vi "Diagnostics - Tool.vi"() -> ()   [LabVIEW 2025, in "Diagnostics Workspace Tool.lvlib"]
uses:
  Diagnostics Workspace Tool.lvlib
  Addon/Addon Shared/Types/Command.New.ctl
  NationalInstruments.VeriStand.SystemStorage
  SubModules/CAN-Streaming-Support/Source/Addon/Addon Shared/Types/Direction Filter.ctl
  SubModules/CAN-Streaming-Support/Source/Addon/Addon Shared/Types/Type Filter.ctl
  Workspace Shared/Types/Workspace.State.ctl
  Workspace Shared/Types/UI.Refs.ctl
  <vilib>/NI VeriStand/Display Template Support/DisplayTemplateSupport.llb/enum_Display Template Handler Minimal To Workspace.ctl
  Workspace Shared/Types/Workspace.SavedState.ctl
  <vilib>/NI VeriStand/Execution/Workspace/WorkspaceAPI.ctl
  <vilib>/NI VeriStand/Display Template Support/DisplayTemplateSupport.llb/enum_Display Template Handler Minimal To Widget Msg.ctl
  <vilib>/NI VeriStand/Execution/Workspace/SystemStateRegEventRef.ctl
  <vilib>/NI VeriStand/Execution/Workspace/Target State Info.ctl
  <vilib>/NI VeriStand/Execution/Workspace/Target State.ctl
  <vilib>/NI VeriStand/Execution/Workspace/SystemStateEventRef.ctl
  Addon/Addon Shared/Types/Protocol.ctl
  SubModules/CAN-Streaming-Support/Source/UIs/Workspace Shared/Types/Host Stream Queue Refs.ctl
  SubModules/CAN-Streaming-Support/Source/UIs/Workspace Shared/Types/Host Stream Queue Type.ctl
  SubModules/CAN-Streaming-Support/Source/UIs/Workspace Shared/Types/Host Stream Queue Command.ctl
  <vilib>/xnet/xnet.llb/XNET Frame CAN.ctl
  <vilib>/xnet/xnet.llb/XNET Frame Type CAN.ctl
  Addon/Addon Shared/Types/Transport.ctl
  SubModules/CAN-Streaming-Support/Source/UIs/Workspace Shared/Types/Host Stream Engine Parameters.ctl
  SubModules/CAN-Streaming-Support/Source/Addon/Addon Shared/Types/Filter Parameters.ctl
  Addon/Addon Shared/Types/Command.ReadDTC.ctl
  Addon/Addon Shared/Types/DTC.Descriptor.Override.ctl
  <vilib>/Utility/miscctls.llb/LVRowAndColumnUnsignedTypeDef.ctl
  <vilib>/Utility/error.llb/Trim Whitespace.vi
  <vilib>/dlg_ctls.llb/Space Constant.vi
  SubModules/CAN-Streaming-Support/Source/UIs/Workspace Shared/SubVIs/Create Host Stream Refs.vi
  SubModules/CAN-Streaming-Support/Source/UIs/Workspace Shared/SubVIs/Read Host Stream.vi
  SubModules/CAN-Streaming-Support/Source/UIs/Workspace Shared/SubVIs/Cleanup Host Stream.vi
  SubModules/CAN-Streaming-Support/Source/UIs/Workspace Shared/SubVIs/Create Bus Log File.vi
  SubModules/CAN-Streaming-Support/Source/UIs/Workspace Shared/SubVIs/Write to Bus Log File.vi
  SubModules/CAN-Streaming-Support/Source/UIs/Workspace Shared/SubVIs/Convert BIN to TXT File.vi
  SubModules/CAN-Streaming-Support/Source/UIs/Workspace Shared/SubVIs/Get Next Bus Engine State.vi
  SubModules/CAN-Streaming-Support/Source/UIs/Workspace Shared/SubVIs/Get Engine Trigger State.vi
  SubModules/CAN-Streaming-Support/Source/UIs/Workspace Shared/SubVIs/Get Next Log Engine State.vi
  <vilib>/Utility/error.llb/Trim Whitespace One-Sided.vi
  SubModules/CAN-Streaming-Support/Source/UIs/Workspace Shared/SubVIs/Process CAN Data.vi
  SubModules/CAN-Streaming-Support/Source/UIs/Workspace Shared/SubVIs/Process CAN State.vi
  SubModules/CAN-Streaming-Support/Source/UIs/Workspace Shared/SubVIs/Convert Frame Array to String Array.vi
  SubModules/CAN-Streaming-Support/Source/UIs/Workspace Shared/SubVIs/Convert Time to UTC String.vi
  <userlib>/_OpenG.lib/array/array.llb/Sort Array__ogtk.vi
  <userlib>/_OpenG.lib/array/array.llb/Sort 2D Array (String)__ogtk.vi
  <vilib>/Utility/libraryn.llb/Check if File or Folder Exists.vi
  <vilib>/Utility/libraryn.llb/Get File Extension.vi
  Addon/Addon Shared/SubVIs/Constants.vi
  <vilib>/NI VeriStand/Execution/Workspace/NI VeriStand - Get Multiple Channel Values.vi
  <vilib>/NI VeriStand/Execution/Workspace/NI VeriStand - Set Single Channel Value.vi
  Workspace Shared/Diagnostics Workspace Shared.lvlib
  APIs/Host Automation API/Diagnostics Host Automation API.lvlib
  Addon/Addon Shared/Diagnostics Addon Shared.lvlib
  <vilib>/NI VeriStand/Execution/Workspace/NI_VS Workspace ExecutionAPI.lvlib
  SubModules/CAN-Streaming-Support/Source/UIs/Workspace Shared/CAN Stream Support Workspace Shared.lvlib
  SubModules/CAN-Streaming-Support/Source/Addon/Addon Shared/CAN Stream Support Shared.lvlib
  NationalInstruments.VeriStand.ClientAPI
panel:
  out "Device":string
  in  "Tab Control":enum32{"Cmd", "Raw", "Read DTCs", "Bus Stream"}(tab)
  out "Time Stamp":timestamp
  out "Comm Connected?":bool
  in  "Send Cmd":bool
  out "VeriStand Error":i64 format="%.0x"
  out "Success?":bool
  in  "Cmd":T1
  in  "Clear Raw":bool
  in  "Send Raw":bool
  out "Raw VeriStand Error":errorcluster
  out "Raw Error Byte":u8 format="%.0x"
  in  "Response Required?":bool
  out "Raw Resp":u8[](array[numeric]) format="%.0x"
  in  "Raw Cmd":u8[](array[numeric]) format="%.0x"
  in  "DTC":u32
  in  "Status":u32
  in  "Failure":u32
  in  "Override Byte Lengths":bool
  in  "Extension":u32 format="%.0x"
  in  "Mask":u32 format="%.0x"
  in  "Mode":u32 format="%.0x"
  in  "Hex":bool=TRUE
  in  "DTCs":string(tree)
  in  "Read DTCs":bool
  in  "Reset Filter":bool
  in  "Host Filter":bool
  in  "Filter IDs":string caption="Filter IDs (format = x<ID>, comma separated, ID x0 = Bus Error)"
  in  "Clear History":bool
  in  "Type Filter":T2
  out "Table Control":string[][](table)
  in  "Enable Stream":bool
  in  "Pause":bool
  in  "Sort By ID":bool
  out "Stream Connected":bool
  out "Status":string
  in  "Direction Filter":T3
  in  "Log":bool
  in  "NIVS.Gateway IP Address":string
  in  "NIVS.System Definition Root":refnum<k24>
  in  "NIVS.Workspace Event":refnum<event-registration>
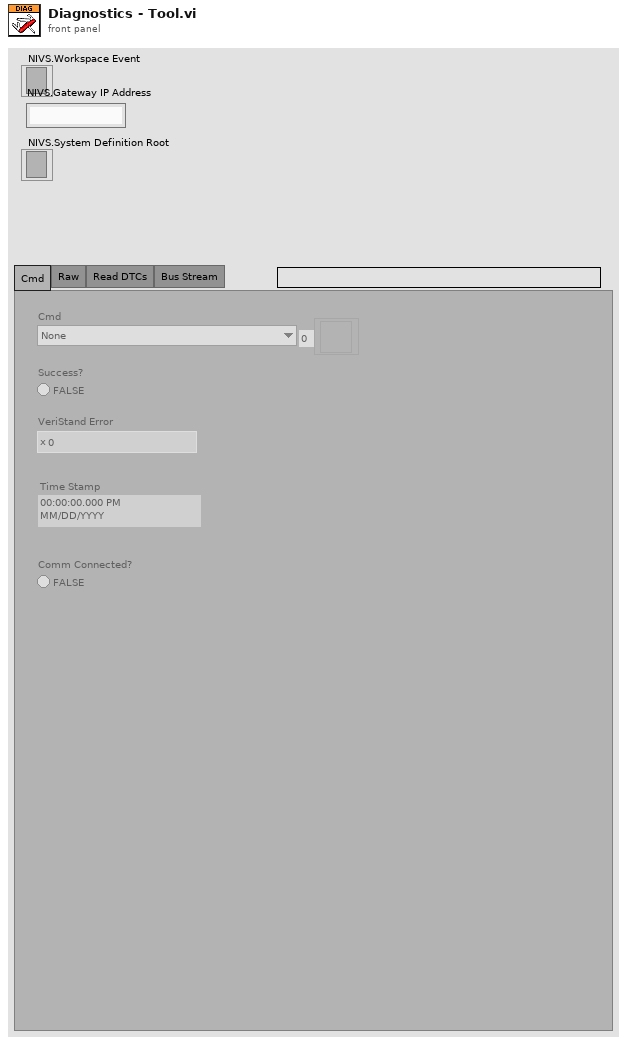
[diagram p1: front panel]
types:
  T1 = typedef "Diagnostics Addon Shared.lvlib/Command.New.ctl" = enum8{"None", "Clear Status Channels", "Read All DIDs", "Read All PIDs", "Configure and Start DPIDs", "Stop DPIDs"}
  T2 = typedef "CAN Stream Support Shared.lvlib/Type Filter.ctl" = enum16{"All", "CAN Data", "CAN Remote", "CAN Bus Error", "CAN 2.0 Data", "CAN FD Data", "CAN FD+BRS Data", "J1939 Data", "Delay", "Log Trigger", "Start Trigger"}
  T3 = typedef "CAN Stream Support Shared.lvlib/Direction Filter.ctl" = enum16{"Tx/Rx", "Rx", "Tx"}
  T4 = typedef "Diagnostics Workspace Shared.lvlib/Workspace.State.ctl" = cluster{"UI.Refs":T5, "Data.PreviousValues":dbl[], "Data.Read":string[], "CachedData.UserEvent":refnum<user-event>, "CachedData":T6, "Addon.Connected?":bool, "NIVS.SysDef":path, "NIVS.SysDefRoot":refnum<k24>, "NIVS.Workspace":T7, "NIVS.UserEventRefs":cluster{"Event Registration Refnum":refnum<event-registration>, "SystemChangeEventRef":T8, "NIVS.Workspace Event":refnum<event-registration>}, "NIVS.SystemStateRefs":T9, "NIVS.LaunchRef":refnum<user-event>, "Data.PendingChange?":bool, "Command.Channel":string, "Diagnostic Protocol":T10, "Channels.Found":bool, "Command.Connect":string, "Mode.Tool?":bool, "Stream.Qs":T11, "Transport Layer":T12}
  T5 = typedef "Diagnostics Workspace Shared.lvlib/UI.Refs.ctl" = cluster{"Cmd":refnum<vi>, "Success?":refnum<vi>, "VeriStandError":refnum<vi>, "CAN Connected?":refnum<vi>, "DTC":refnum<vi>, "Status":refnum<vi>, "Failure":refnum<vi>, "Override Byte Lengths":refnum<vi>, "Response Required?":refnum<vi>, "Send":refnum<vi>, "Clear":refnum<vi>, "Send Raw":refnum<vi>, "Read DTCs":refnum<vi>, "Raw Cmd":refnum<vi>, "Extension":refnum<vi>, "Mode":refnum<vi>, "Mask":refnum<vi>, "Hex":refnum<vi>, "Raw Resp":refnum<vi>, "Raw Error Byte":refnum<vi>, "Raw VeriStand Error":refnum<vi>, "DTCs":refnum<vi>, "Time Stamp":refnum<vi>, "Device":refnum<vi>, "Pause":refnum<vi>, "Table Control":refnum<vi>, "Sort By ID":refnum<vi>, "Streaming Connected":refnum<vi>, "Enable Stream":refnum<vi>, "CAN State":refnum<vi>, "Direction Filter":refnum<vi>, "Type Filter":refnum<vi>, "Clear History":refnum<vi>, "Filter IDs":refnum<vi>, "Filter Location":refnum<vi>, "Reset Filter":refnum<vi>, "Log":refnum<vi>}
  T6 = typedef "Diagnostics Workspace Shared.lvlib/Workspace.SavedState.ctl" = cluster{"CD Path":string, "CD IP":string}
  T7 = typedef "NI_VS Workspace ExecutionAPI.lvlib/WorkspaceAPI.ctl" = refnum<k24>
  T8 = typedef "NI_VS Workspace ExecutionAPI.lvlib/SystemStateRegEventRef.ctl" = refnum<event-registration>
  T9 = typedef "NI_VS Workspace ExecutionAPI.lvlib/SystemStateEventRef.ctl" = cluster{"CustDatRef":refnum<user-event>, "EvtRef":refnum<k27>, "Target State User Event":refnum<user-event>}
  T10 = typedef "Diagnostics Addon Shared.lvlib/Protocol.ctl" = enum16{"GMLAN", "KWP-2000", "UDS", "User-Defined"}
  T11 = typedef "CAN Stream Support Workspace Shared.lvlib/Host Stream Queue Refs.ctl" = cluster{"Cmd Q":refnum<queue>, "XNET Frames":refnum<queue>}
  T12 = typedef "Diagnostics Addon Shared.lvlib/Transport.ctl" = enum16{"ISO TP - Normal Mode", "ISO TP - Mixed Mode", "VW TP 2.0", "Diagnostics on IP", "ISO TP LIN"}
  T13 = typedef "enum_Display Template Handler Minimal To Workspace.ctl" = cluster{"Operation":enum16{"SetCustomData", "DeleteItem"}, "Data":variant}
  T14 = typedef "Diagnostics Addon Shared.lvlib/Command.ReadDTC.ctl" = cluster{"Extension":u32, "Mask":u32, "Mode/Status":u32, "Byte Lengths":T15}
  T15 = typedef "Diagnostics Addon Shared.lvlib/DTC.Descriptor.Override.ctl" = cluster{"Override":bool, "DTC":u32, "Status":u32, "Failure":u32}
  T16 = typedef "CAN Stream Support Shared.lvlib/Filter Parameters.ctl" = cluster{"ID Filters":u32[], "Direction Filter":T3, "Type Filter":T2}
  T17 = typedef "LVRowAndColumnUnsignedTypeDef.ctl" = cluster{"Row":u32, "Column":u32}
  T18 = cluster{"Event Registration Refnum":refnum<event-registration>, "SystemChangeEventRef":T8, "NIVS.Workspace Event":refnum<event-registration>}
  T19 = typedef "enum_Display Template Handler Minimal To Widget Msg.ctl" = enum16{"Stop", "LaunchConfigDialog"}
  T20 = enum8{"Enabled", "Disabled", "Disabled and Grayed Out"}
  T21 = typedef "Diagnostics Addon Shared.lvlib/HostAutomation.Ref.ctl" = cluster{"TCP Comm":T22, "DTCs":T24}
  T22 = typedef "NI STM.lvlib/TCP Connection Info.ctl" = cluster{"connection ID":refnum<k5>, "meta data":T23[]}
  T23 = typedef "NI STM.lvlib/MetaDataElement.ctl" = string
  T24 = typedef "Diagnostics Addon Shared.lvlib/DTC.Codes.ctl" = cluster{"Value.Code":dbl[], "Value.String":string[], "Value.J2012String":string[], "Status.Code":dbl[], "Status.String":string[]}
  T25 = cluster{"resp":u8[], "error code":u8, "error out":errorcluster}
  T26 = typedef "Diagnostics Addon Shared.lvlib/Command.ReadDTC.DTCs.ctl" = cluster{"Timestamp":dbl, "DTC":dbl, "J2012 String":string, "DTC String":string, "Status":dbl, "Status String":string, "Add Data":dbl}
  T27 = typedef "CAN Stream Support Workspace Shared.lvlib/Host Stream Engine Parameters.ctl" = cluster{"Host Filter":bool, "Filter Parameters":T16, "Sort By ID":bool, "Pause":bool, "Clear History":bool, "Log":bool}
  T28 = typedef "CAN Stream Support Workspace Shared.lvlib/Host Stream Data.ctl" = cluster{"Connected":bool, "Bus Data Update":bool, "Bus Data":string[][], "Bus Status":string, "Bus Warning":bool, "Log Status":string}
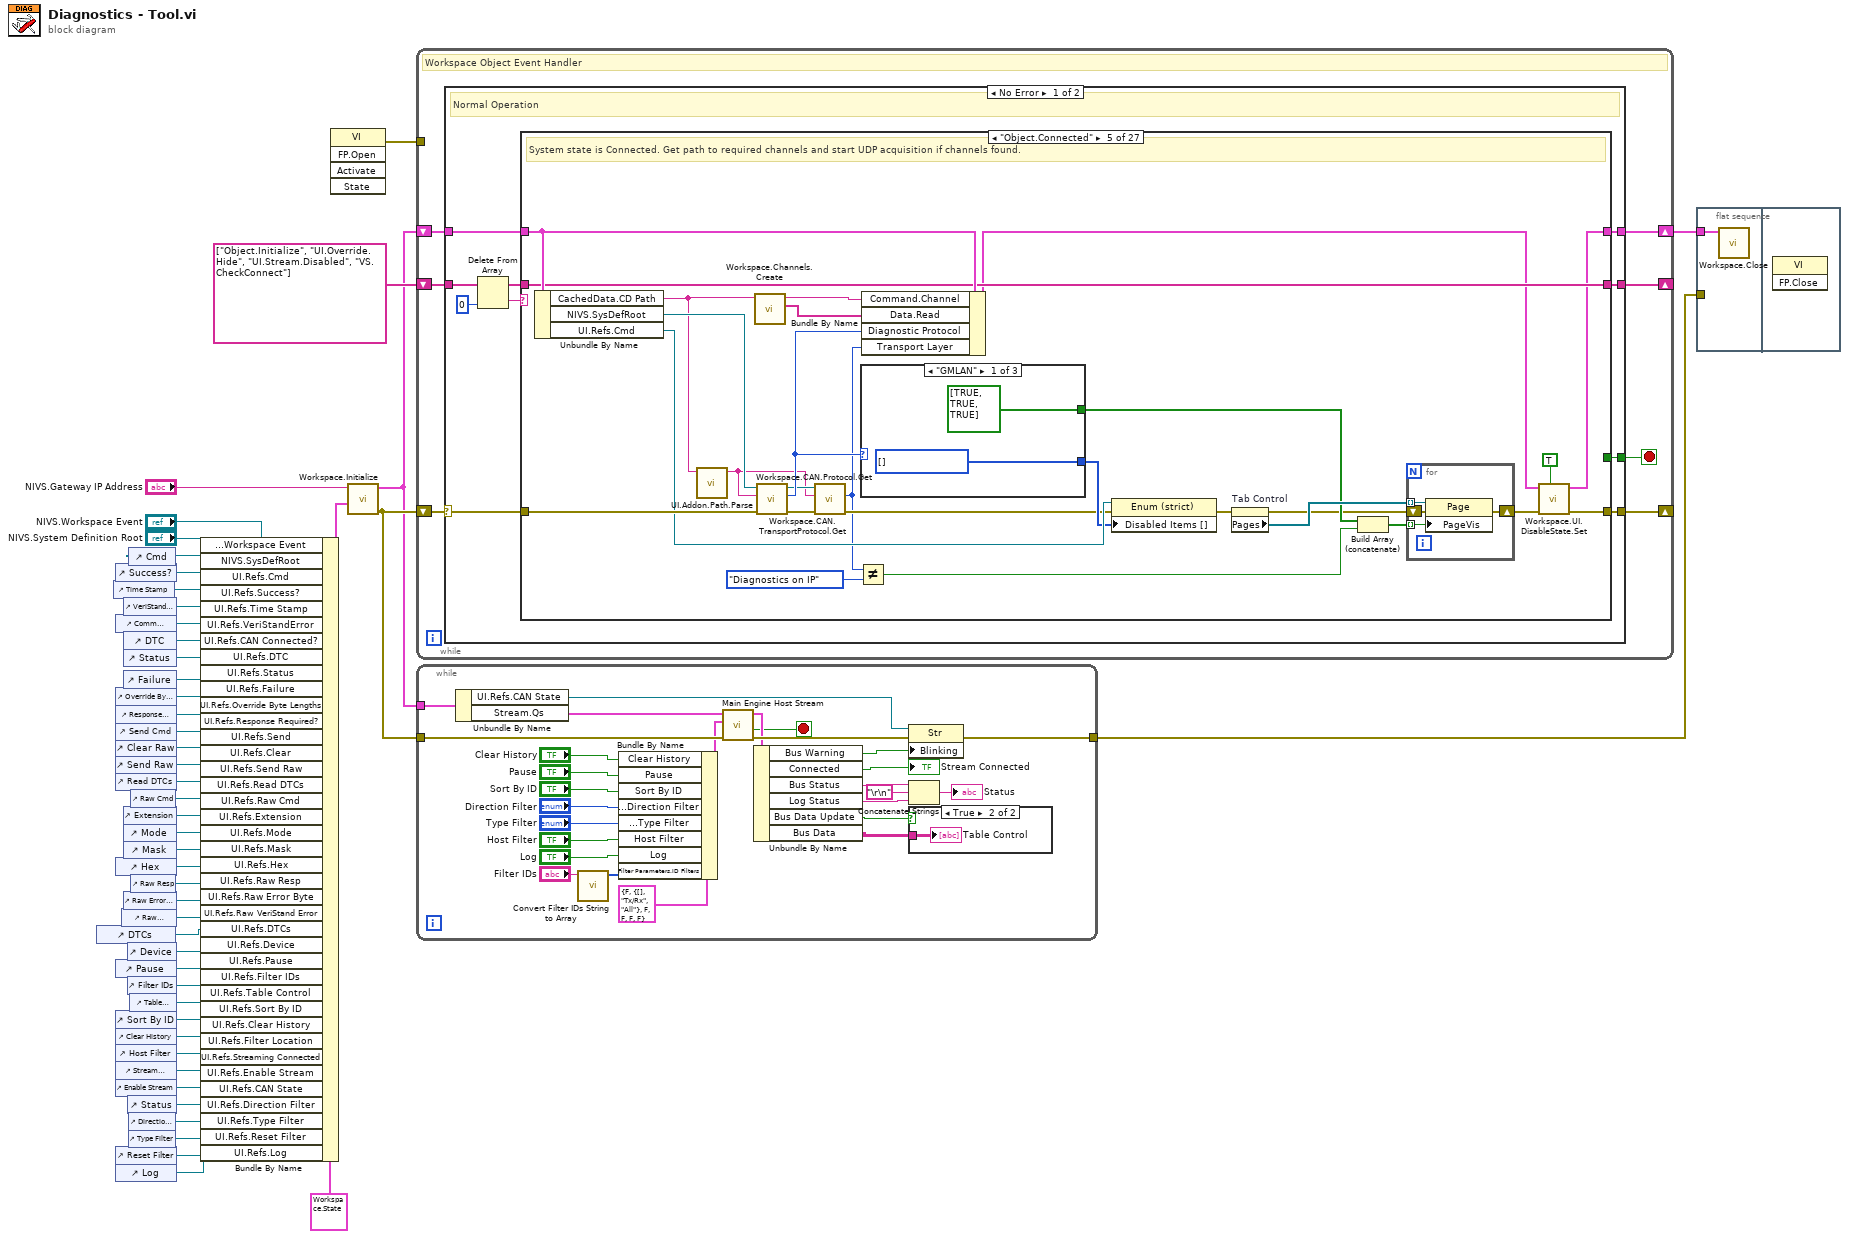
[diagram p0: block diagram]
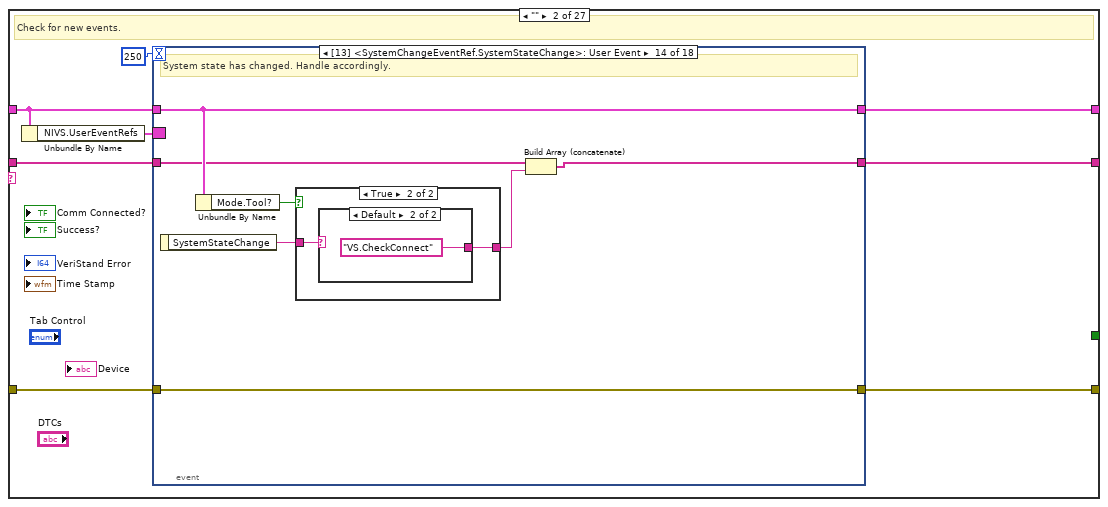
[diagram p4: hidden frame]
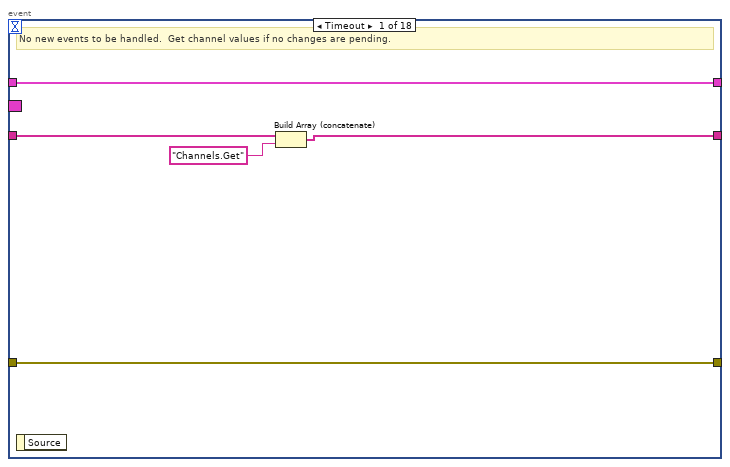
[diagram p5: hidden frame]
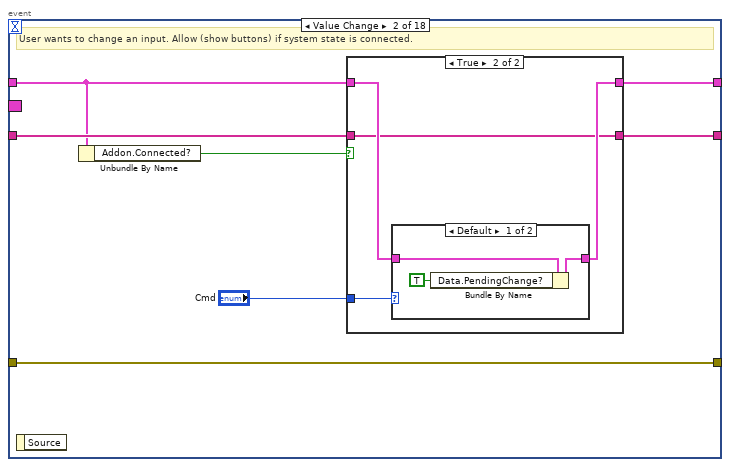
[diagram p6: hidden frame]
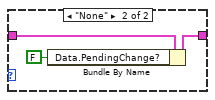
[diagram p8: hidden frame]
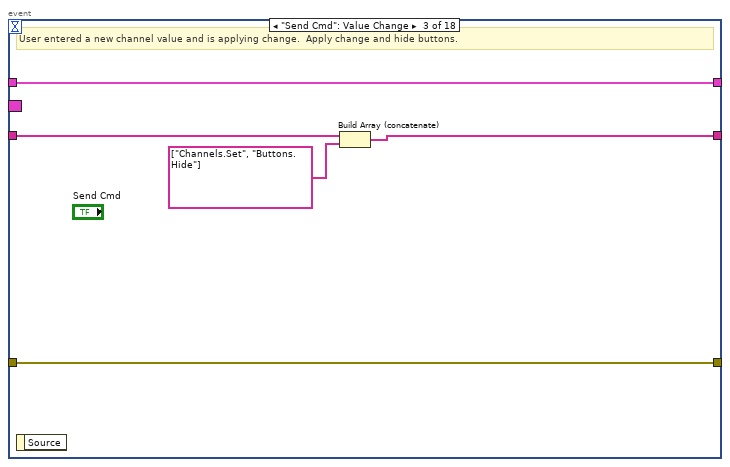
[diagram p9: hidden frame]
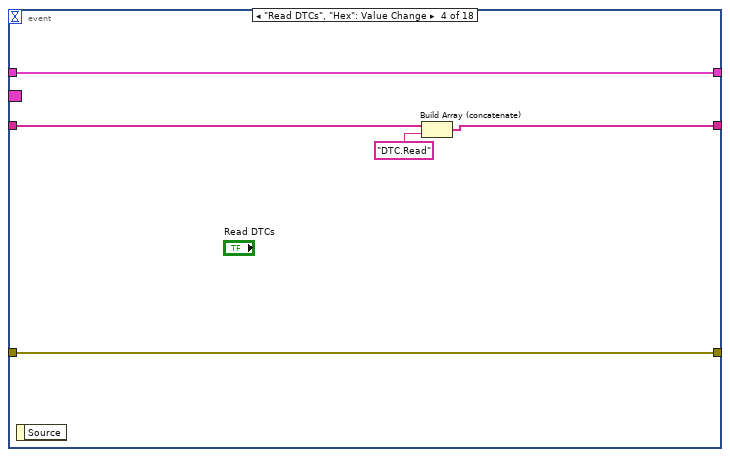
[diagram p10: hidden frame]
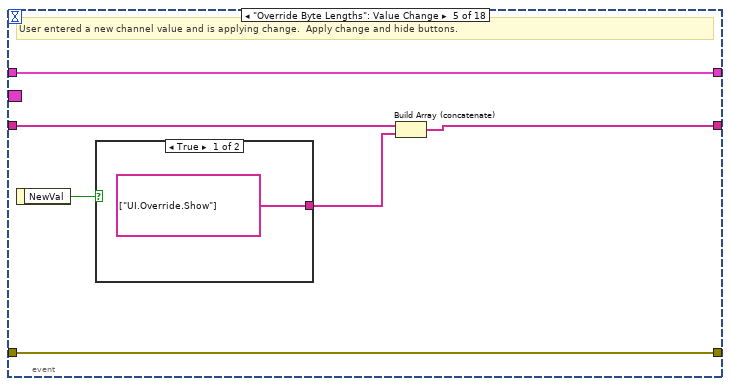
[diagram p11: hidden frame]
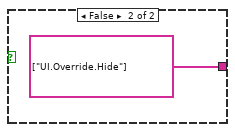
[diagram p12: hidden frame]
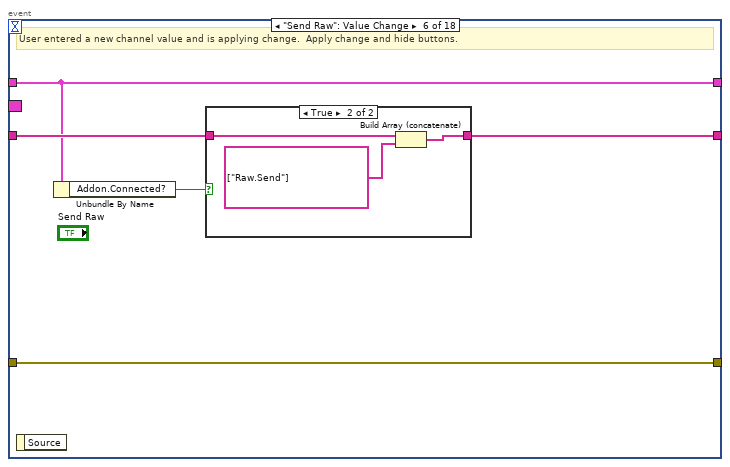
[diagram p13: hidden frame]
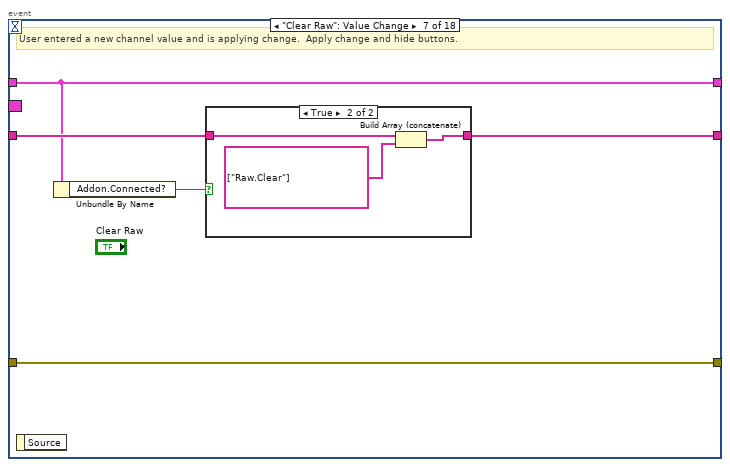
[diagram p15: hidden frame]
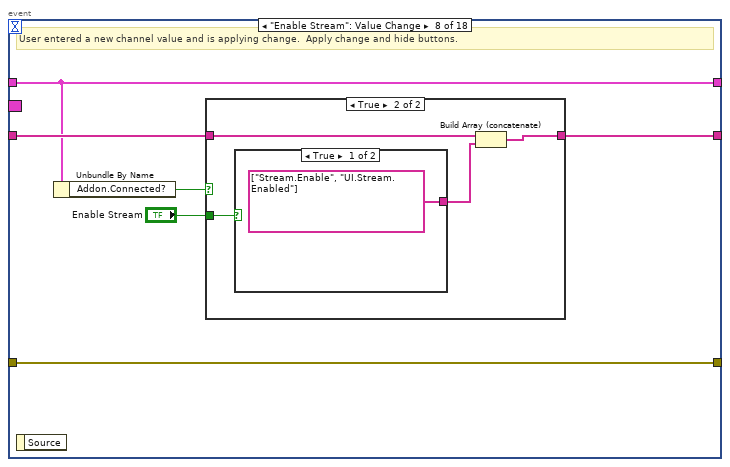
[diagram p17: hidden frame]
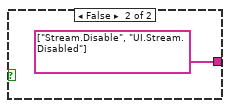
[diagram p19: hidden frame]
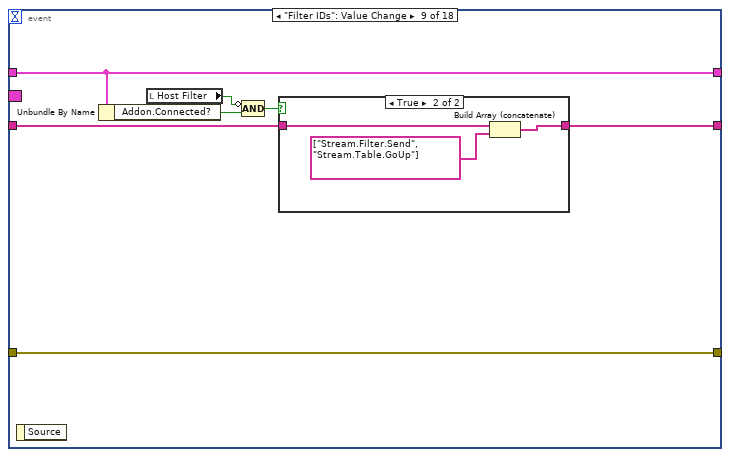
[diagram p20: hidden frame]
diagram:
  n1 = control-ref of="DTCs"() -> (w23:refnum<vi>)
  n2 = control-ref of="Time Stamp"() -> (w18:refnum<vi>)
  n3 = control-ref of="Success?"() -> (w44:refnum<vi>)
  n4 = control-ref of="Comm Connected?"() -> (w43:refnum<vi>)
  n5 = control-ref of="Override Byte Lengths"() -> (w39:refnum<vi>)
  n6 = control-ref of="Response Required?"() -> (w33:refnum<vi>)
  n7 = control-ref of="Send Cmd"() -> (w32:refnum<vi>)
  n8 = control-ref of="Clear Raw"() -> (w31:refnum<vi>)
  n9 = control-ref of="Send Raw"() -> (w30:refnum<vi>)
  n10 = control-ref of="Read DTCs"() -> (w29:refnum<vi>)
  n11 = control-ref of="Hex"() -> (w24:refnum<vi>)
  n12 = control-ref of="Pause"() -> (w16:refnum<vi>)
  n13 = control-ref of="Sort By ID"() -> (w14:refnum<vi>)
  n14 = control-ref of="Clear History"() -> (w4:refnum<vi>)
  n15 = control-ref of="Host Filter"() -> (w3:refnum<vi>)
  n16 = control-ref of="Stream Connected"() -> (w13:refnum<vi>)
  n17 = control-ref of="Enable Stream"() -> (w12:refnum<vi>)
  n18 = control-ref of="Reset Filter"() -> (w2:refnum<vi>)
  n19 = control-ref of="Log"() -> (w1:refnum<vi>)
  n20 = control-ref of="Raw VeriStand Error"() -> (w22:refnum<vi>)
  n21 = control-ref of="VeriStand Error"() -> (w45:refnum<vi>)
  n22 = control-ref of="DTC"() -> (w42:refnum<vi>)
  n23 = control-ref of="Status"() -> (w41:refnum<vi>)
  n24 = control-ref of="Failure"() -> (w40:refnum<vi>)
  n25 = control-ref of="Extension"() -> (w27:refnum<vi>)
  n26 = control-ref of="Mode"() -> (w26:refnum<vi>)
  n27 = control-ref of="Mask"() -> (w25:refnum<vi>)
  n28 = control-ref of="Raw Error Byte"() -> (w21:refnum<vi>)
  n29 = control-ref of="Device"() -> (w17:refnum<vi>)
  n30 = control-ref of="Filter IDs"() -> (w5:refnum<vi>)
  n31 = control-ref of="Status"() -> (w11:refnum<vi>)
  n32 = control-ref of="Cmd"() -> (w19:refnum<vi>)
  n33 = control-ref of="Direction Filter"() -> (w7:refnum<vi>)
  n34 = control-ref of="Type Filter"() -> (w6:refnum<vi>)
  n35 = control-ref of="Table Control"() -> (w15:refnum<vi>)
  n36 = control-ref of="Raw Cmd"() -> (w28:refnum<vi>)
  n37 = control-ref of="Raw Resp"() -> (w20:refnum<vi>)
  n38 = Bundle By Name(cluster=T4 {"UI.Refs"={"Cmd"=refnum, "Success?"=refnum, "VeriStandError"=refnum, "CAN Connected?"=refnum, "DTC"=refnum, "Status"=refnum, "Failure"=refnum, "Override Byte Lengths"=refnum, "Response Required?"=refnum, "Send"=refnum, "Clear"=refnum, "Send Raw"=refnum, "Read DTCs"=refnum, "Raw Cmd"=refnum, "Extension"=refnum, "Mode"=refnum, "Mask"=refnum, "Hex"=refnum, "Raw Resp"=refnum, "Raw Error Byte"=refnum, "Raw VeriStand Error"=refnum, "DTCs"=refnum, "Time Stamp"=refnum, "Device"=refnum, "Pause"=refnum, "Table Control"=refnum, "Sort By ID"=refnum, "Streaming Connected"=refnum, "Enable Stream"=refnum, "CAN State"=refnum, "Direction Filter"=refnum, "Type Filter"=refnum, "Clear History"=refnum, "Filter IDs"=refnum, "Filter Location"=refnum, "Reset Filter"=refnum, "Log"=refnum}, "Data.PreviousValues"=[], "Data.Read"=[], "CachedData.UserEvent"=refnum, "CachedData"={"CD Path"="", "CD IP"=""}, "Addon.Connected?"=FALSE, "NIVS.SysDef"=path "", "NIVS.SysDefRoot"=refnum, "NIVS.Workspace"=refnum, "NIVS.UserEventRefs"={"Event Registration Refnum"=refnum, "SystemChangeEventRef"=refnum, "NIVS.Workspace Event"=refnum}, "NIVS.SystemStateRefs"={"CustDatRef"=refnum, "EvtRef"=refnum, "Target State User Event"=refnum}, "NIVS.LaunchRef"=refnum, "Data.PendingChange?"=FALSE, "Command.Channel"="", "Diagnostic Protocol"=enum."GMLAN", "Channels.Found"=FALSE, "Command.Connect"="", "Mode.Tool?"=FALSE, "Stream.Qs"={"Cmd Q"=refnum, "XNET Frames"=refnum}, "Transport Layer"=enum."Diagnostics on IP"}, "NIVS.UserEventRefs.NIVS.Workspace Event"="NIVS.Workspace Event", "NIVS.SysDefRoot"="NIVS.System Definition Root", "UI.Refs.Cmd"=w19, "UI.Refs.Success?"=w44, "UI.Refs.Time Stamp"=w18, "UI.Refs.VeriStandError"=w45, "UI.Refs.CAN Connected?"=w43, "UI.Refs.DTC"=w42, "UI.Refs.Status"=w41, "UI.Refs.Failure"=w40, "UI.Refs.Override Byte Lengths"=w39, "UI.Refs.Response Required?"=w33, "UI.Refs.Send"=w32, "UI.Refs.Clear"=w31, "UI.Refs.Send Raw"=w30, "UI.Refs.Read DTCs"=w29, "UI.Refs.Raw Cmd"=w28, "UI.Refs.Extension"=w27, "UI.Refs.Mode"=w26, "UI.Refs.Mask"=w25, "UI.Refs.Hex"=w24, "UI.Refs.Raw Resp"=w20, "UI.Refs.Raw Error Byte"=w21, "UI.Refs.Raw VeriStand Error"=w22, "UI.Refs.DTCs"=w23, "UI.Refs.Device"=w17, "UI.Refs.Pause"=w16, "UI.Refs.Filter IDs"=w5, "UI.Refs.Table Control"=w15, "UI.Refs.Sort By ID"=w14, "UI.Refs.Clear History"=w4, "UI.Refs.Filter Location"=w3, "UI.Refs.Streaming Connected"=w13, "UI.Refs.Enable Stream"=w12, "UI.Refs.CAN State"=w11, "UI.Refs.Direction Filter"=w7, "UI.Refs.Type Filter"=w6, "UI.Refs.Reset Filter"=w2, "UI.Refs.Log"=w1) -> (w46:T4)
  n39 = invoke class="VI" method="FP.Open"() -> (error out=w37:errorcluster)  [unwired: 5 in, 4 out]
  n40 = call "Workspace.Initialize.vi"("State Variables in"=w46, "NIVS.Gateway IP Address"="NIVS.Gateway IP Address") -> ("error out"=w10:errorcluster, "State Variables out"=w9:T4)  [unwired: 8 in]
  n41 = while {
    shift-right: [w53] -> _
    shift-left: string[] ["Object.Initialize", "UI.Override.Hide", "UI.Stream.Disabled", "VS.CheckConnect"] -> [w54]
    shift-right: [w51] -> w36
    shift-left: w9 -> [w50]
    shift-right: [w52] -> _
    shift-left: w10 -> [w49]
    tunnel: w37 -> [_]
    stop <- w55 stop-if-true
    # "Workspace Object Event Handler"
    n42 = case shown="No Error" w49 {
      selector: w49 -> [w56 w622]
      tunnel: [w65 _] -> w55
      tunnel: w54 -> [w63 w629]
      tunnel: [w60 w629] -> w53
      tunnel: [w59 w620] -> w52
      tunnel: [w58 w628] -> w51
      tunnel: w50 -> [w57 w628]
      frame No Error {
        # "Normal Operation"
        n43 = Delete From Array(array=w63, index=0) -> (deleted portion=w62:string, array with subset deleted=w61:string[])  [unwired: 1 in]
        n44 = case shown="\"Object.Connected\"" w62 {
          tunnel: [_ _ _ _ _ _ _ TRUE _ _ _ _ _ _ _ _ _ _ _ _ _ _ _ _ _ _ _] -> w65
          tunnel: [w68 w75 w270 w277 w318 w335 w341 w362 w369 w382 w405 w423 w436 w444 w458 w471 w484 w507 w511 w536 w545 w563 w575 w592 w608 w614 w619] -> w60
          tunnel: w56 -> [w67 w73 w271 w283 w315 w333 w346 w359 w368 w380 w404 w417 w430 w442 w455 w469 w481 w506 w510 w515 w544 w556 w568 w585 w599 w609 w615]
          tunnel: w61 -> [w68 w74 w270 w276 w318 w335 w340 w362 w369 w382 w405 w423 w436 w444 w458 w471 w484 w507 w511 w536 w545 w563 w575 w592 w608 w614 w619]
          tunnel: w57 -> [w66 w69 w267 w281 w319 w332 w338 w358 w365 w375 w402 w422 w435 w441 w457 w470 w483 w503 w509 w535 w542 w559 w571 w588 w602 w613 w618]
          tunnel: [w67 w72 w263 w283 w304 w330 w345 w360 w368 w379 w403 w416 w429 w443 w446 w468 w473 w506 w510 w513 w543 w556 w568 w585 w599 w610 w616] -> w59
          tunnel: [w66 w71 w267 w280 w302 w331 w339 w358 w365 w378 w401 w422 w435 w441 w457 w470 w483 w503 w509 w535 w542 w559 w571 w588 w602 w613 w618] -> w58
          frame Default {
            # "Do nothing."
          }
          frame "" {
            # "Check for new events."
            n45 = Unbundle By Name(w69) -> ("NIVS.UserEventRefs"=w70:T18)
            n46 = event shown="[13] <SystemChangeEventRef.SystemStateChange>: User Event" {
              selector: w70 -> [_ _ _ _ _ _ _ _ _ _ _ _ _ _ _ _ _ _]
              dyn-events: _ -> [_ _ _ _ _ _ _ _ _ _ _ _ _ _ _ _ _ _]
              timeout: 250 -> [_ _ _ _ _ _ _ _ _ _ _ _ _ _ _ _ _ _]
              tunnel: [w77 w86 w101 w106 w114 w121 w130 w140 w155 w166 w175 w185 w198 w208 w221 w237 w251 w258] -> w75
              tunnel: w74 -> [w80 w87 w102 w107 w115 w122 w131 w141 w154 w165 w174 w184 w197 w210 w220 w236 w252 w259]
              tunnel: w73 -> [w81 w82 w105 w110 w116 w123 w132 w142 w156 w167 w176 w186 w199 w207 w228 w235 w255 w261]
              tunnel: [w81 w82 w105 w110 w116 w123 w132 w142 w156 w167 w176 w186 w199 w207 w228 w235 w255 w261] -> w72
              tunnel: [w78 w88 w104 w109 w113 w120 w129 w139 w153 w164 w173 w183 w196 w212 w227 w233 w254 w260] -> w71
              tunnel: w69 -> [w78 w85 w104 w109 w113 w120 w129 w139 w153 w164 w173 w183 w196 w212 w227 w234 w254 w260]
              event Timeout {
                # "No new events to be handled.  Get channel values if no changes are pending."
                n47 = event-data() -> ()  [unwired: 2 out]
                n48 = Build Array (concatenate)(w80, "Channels.Get") -> (w77:string[])
              }
              event Value Change {
                # "User wants to change an input. Allow (show buttons) if system state is connected."
                n49 = event-data() -> ()  [unwired: 2 out]
                n50 = Unbundle By Name(w85) -> ("Addon.Connected?"=w84:bool)
                n51 = case shown="True" w84 {
                  tunnel: w85 -> [w89 w94]
                  tunnel: [w89 w93] -> w88
                  tunnel: w87 -> [w90 w92]
                  tunnel: [w90 w92] -> w86
                  tunnel: "Cmd" -> [_ w91]
                  frame False {
                  }
                  frame True {
                    n52 = case shown="Default" w91 {
                      tunnel: w94 -> [w96 w99]
                      tunnel: [w95 w98] -> w93
                      frame Default {
                        n53 = Bundle By Name(cluster=w96, "Data.PendingChange?"=TRUE ("Pending Change?")) -> (w95:T4)
                      }
                      frame "None" {
                        n54 = Bundle By Name(cluster=w99, "Data.PendingChange?"=FALSE ("Pending Change?")) -> (w98:T4)
                      }
                    }
                  }
                }
              }
              event "Send Cmd": Value Change {
                # "User entered a new channel value and is applying change.  Apply change and hide buttons."
                n55 = event-data() -> ()  [unwired: 2 out]
                n56 = Build Array (concatenate)(w102, string[] ["Channels.Set", "Buttons.Hide"]) -> (w101:string[])
              }
              event "Read DTCs", "Hex": Value Change {
                n57 = event-data() -> ()  [unwired: 2 out]
                n58 = Build Array (concatenate)(w107, "DTC.Read") -> (w106:string[])
              }
              event "Override Byte Lengths": Value Change {
                # "User entered a new channel value and is applying change.  Apply change and hide buttons."
                n59 = event-data() -> ("NewVal"=w111:bool)  [unwired: 1 out]
                n60 = case shown="True" w111 {
                  tunnel: [string[] ["UI.Override.Show"] string[] ["UI.Override.Hide"]] -> w112
                  frame True {
                  }
                  frame False {
                  }
                }
                n61 = Build Array (concatenate)(w115, w112) -> (w114:string[])
              }
              event "Send Raw": Value Change {
                # "User entered a new channel value and is applying change.  Apply change and hide buttons."
                n62 = event-data() -> ()  [unwired: 2 out]
                n63 = Unbundle By Name(w120) -> ("Addon.Connected?"=w119:bool)
                n64 = case shown="True" w119 {
                  tunnel: w122 -> [w124 w126]
                  tunnel: [w124 w125] -> w121
                  frame False {
                  }
                  frame True {
                    n65 = Build Array (concatenate)(w126, string[] ["Raw.Send"]) -> (w125:string[])
                  }
                }
              }
              event "Clear Raw": Value Change {
                # "User entered a new channel value and is applying change.  Apply change and hide buttons."
                n66 = event-data() -> ()  [unwired: 2 out]
                n67 = Unbundle By Name(w129) -> ("Addon.Connected?"=w128:bool)
                n68 = case shown="True" w128 {
                  tunnel: w131 -> [w133 w135]
                  tunnel: [w133 w134] -> w130
                  frame False {
                  }
                  frame True {
                    n69 = Build Array (concatenate)(w135, string[] ["Raw.Clear"]) -> (w134:string[])
                  }
                }
              }
              event "Enable Stream": Value Change {
                # "User entered a new channel value and is applying change.  Apply change and hide buttons."
                n70 = event-data() -> ()  [unwired: 2 out]
                n71 = Unbundle By Name(w139) -> ("Addon.Connected?"=w138:bool)
                n72 = case shown="True" w138 {
                  tunnel: w141 -> [w143 w146]
                  tunnel: [w143 w145] -> w140
                  tunnel: "Enable Stream" -> [_ w144]
                  frame False {
                  }
                  frame True {
                    n73 = case shown="True" w144 {
                      tunnel: [string[] ["Stream.Enable", "UI.Stream.Enabled"] string[] ["Stream.Disable", "UI.Stream.Disabled"]] -> w147
                      frame True {
                      }
                      frame False {
                      }
                    }
                    n74 = Build Array (concatenate)(w146, w147) -> (w145:string[])
                  }
                }
              }
              event "Filter IDs": Value Change {
                n75 = event-data() -> ()  [unwired: 2 out]
                n76 = Unbundle By Name(w153) -> ("Addon.Connected?"=w151:bool)
                n77 = local read "Host Filter"() -> (w152:bool)
                n78 = Compound Arithmetic op=AND(invert w152, w151) -> (w150:bool)
                n79 = case shown="True" w150 {
                  tunnel: w154 -> [w157 w161]
                  tunnel: [w158 w160] -> w155
                  frame False {
                    n80 = Build Array (concatenate)(w157, "Stream.Table.GoUp") -> (w158:string[])
                  }
                  frame True {
                    n81 = Build Array (concatenate)(w161, string[] ["Stream.Filter.Send", "Stream.Table.GoUp"]) -> (w160:string[])
                  }
                }
              }
              event "Clear History", "Sort By ID": Value Change {
                n82 = event-data() -> ()  [unwired: 2 out]
                n83 = Unbundle By Name(w164) -> ("Addon.Connected?"=w163:bool)
                n84 = case shown="True" w163 {
                  tunnel: [w168 w171] -> w166
                  tunnel: w165 -> [w168 w170]
                  frame False {
                  }
                  frame True {
                    n85 = Build Array (concatenate)(w170, "Stream.Table.GoUp") -> (w171:string[])
                  }
                }
              }
              event "Reset Filter": Value Change {
                n86 = event-data() -> ()  [unwired: 2 out]
                n87 = Unbundle By Name(w173) -> ("Addon.Connected?"=w172:bool)
                n88 = case shown="True" w172 {
                  tunnel: w174 -> [w177 w179]
                  tunnel: [w177 w178] -> w175
                  frame False {
                  }
                  frame True {
                    n89 = Build Array (concatenate)(w179, string[] ["Stream.Filter.Reset", "Stream.Table.GoUp"]) -> (w178:string[])
                  }
                }
              }
              event "Host Filter": Value Change {
                n90 = event-data() -> ("NewVal"=w181:bool)  [unwired: 1 out]
                n91 = Unbundle By Name(w183) -> ("Addon.Connected?"=w182:bool)
                n92 = case shown="True" w182 {
                  tunnel: w184 -> [w187 w190]
                  tunnel: [w187 w189] -> w185
                  tunnel: w181 -> [_ w188]
                  frame False {
                  }
                  frame True {
                    n93 = case shown="True" w188 {
                      tunnel: [string[] ["Stream.Filter.Send", "Stream.Table.GoUp"] string[] ["Stream.Filter.Clear", "Stream.Table.GoUp"]] -> w191
                      frame False {
                      }
                      frame True {
                      }
                    }
                    n94 = Build Array (concatenate)(w190, w191) -> (w189:string[])
                  }
                }
              }
              event "Log": Value Change {
                n95 = event-data() -> ("NewVal"=w194:bool)  [unwired: 1 out]
                n96 = Unbundle By Name(w196) -> ("Addon.Connected?"=w195:bool)
                n97 = case shown="True" w195 {
                  tunnel: w197 -> [w200 w203]
                  tunnel: [w200 w202] -> w198
                  tunnel: w194 -> [_ w201]
                  frame False {
                  }
                  frame True {
                    n98 = case shown="False" w201 {
                      tunnel: [string[] ["UI.Log.Disabled"] string[] ["UI.Log.Enabled"]] -> w204
                      frame False {
                      }
                      frame True {
                      }
                    }
                    n99 = Build Array (concatenate)(w203, w204) -> (w202:string[])
                  }
                }
              }
              event User Event {
                # "System state has changed. Handle accordingly."
                n100 = event-data() -> ("SystemStateChange"=w211:string)  [unwired: 1 out]
                n101 = Unbundle By Name(w212) -> ("Mode.Tool?"=w213:bool)
                n102 = case shown="True" w213 {
                  tunnel: ["VS.CheckConnect" w216] -> w209
                  tunnel: w211 -> [_ w215]
                  frame False {
                  }
                  frame True {
                    n103 = case shown="Default" w215 {
                      tunnel: ["Object.Exit" "VS.CheckConnect"] -> w216
                      frame "Stop Configuration" {
                      }
                      frame Default {
                      }
                    }
                  }
                }
                n104 = Build Array (concatenate)(w210, w209) -> (w208:string[])
              }
              event User Event {
                n105 = event-data() -> ("Workspace Event"=w222:string)  [unwired: 1 out]
                n106 = Equal?(x=w222, y="Shut Down") -> (x = y?=w223:bool)
                n107 = Equal?(x=w222, y="Disconnect") -> (x = y?=w224:bool)
                n108 = Compound Arithmetic op=OR(w223, w224) -> (w219:bool)
                n109 = case shown="True" w219 {
                  tunnel: [w229 w231] -> w221
                  tunnel: w220 -> [w229 w230]
                  frame False {
                  }
                  frame True {
                    n110 = Build Array (concatenate)(w230, "Object.Exit") -> (w231:string[])
                  }
                }
              }
              event User Event {
                # "Widget event has occurred.  Handle accordingly."
                n111 = event-data() -> ("ToWidgetMessage"=w238:T19)  [unwired: 1 out]
                n112 = case shown="\"LaunchConfigDialog\"" w238 {
                  tunnel: [w240 w243 w249] -> w237
                  tunnel: w236 -> [w240 w244 w250]
                  tunnel: w234 -> [w239 w241 w247]
                  tunnel: [w239 w241 w246] -> w233
                  frame Default {
                    # "Do nothing."
                  }
                  frame "Stop" {
                    # "User exiting workspace or deleting object"
                    n113 = Build Array (concatenate)(w244, "Object.Exit") -> (w243:string[])
                  }
                  frame "LaunchConfigDialog" {
                    # "User wants to configure object"
                    n114 = Build Array (concatenate)(w250, "Object.Configure") -> (w249:string[])
                    n115 = Bundle By Name(cluster=w247, "Data.PendingChange?"=FALSE ("Pending Change?")) -> (w246:T4)
                  }
                }
              }
              event Menu Selection (User) {
                n116 = event-data() -> ("ItemTag"=w253:string)  [unwired: 1 out]
                n117 = Build Array (concatenate)(w252, w253) -> (w251:string[])
              }
              event Panel Close? {
                n118 = event-data() -> ()  [unwired: 5 out]
                n119 = Build Array (concatenate)(w259, "Object.Exit") -> (w258:string[])
                n120 = event-data("Discard?"=TRUE) -> ()  [unwired: 1 in, 1 out]
              }
            }
          }
          frame "Object.Initialize" {
            # "Initialize the workspace Object state variables and UI"
            n121 = invoke on="DTCs" class="Tree (strict)" method="Edit Tree Items.Delete"(error in=w271, "Delete Children"=TRUE ("Delete Children?")) -> (error out=w266:errorcluster)  [unwired: 3 in, 4 out]
            n122 = local write "Tab Control"(0) -> ()
            n123 = Unbundle By Name(w267) -> ("UI.Refs.Filter Location"=w262:refnum<vi>, "UI.Refs.Override Byte Lengths"=w269:refnum<vi>)
            n124 = property class="Bool (strict)"(reference=w269, error in=w266, "Value"=FALSE) -> (error out=w264:errorcluster)  [unwired: 1 out]
            n125 = property class="Bool (strict)"(reference=w262, error in=w264, "Value"=FALSE) -> (error out=w263:errorcluster)  [unwired: 1 out]
          }
          frame "Object.Configure" {
            # "Allow the user to select a control object to display"
            n126 = Unbundle By Name(w281) -> ("NIVS.SysDefRoot"=w275:refnum<k24>, "CachedData.CD Path"=w282:string)
            n127 = call "Workspace.Select.Dialog.vi"("CD Path"=w282, "NIVS.System Definition Root"=w275) -> ("Cancelled?"=w279:bool, "IP Address"=w274:string, "Custom Device Path Out"=w278:string)  [unwired: 7 in]
            n128 = case shown="False" w279 {
              tunnel: w281 -> [w290 w291]
              tunnel: [w289 w291] -> w280
              tunnel: w278 -> [w288 _]
              tunnel: [w286 w292] -> w277
              tunnel: w276 -> [w287 w292]
              tunnel: w274 -> [w284 _]
              frame False {
                # "Queue up required states and cache new controller path"
                n129 = Bundle By Name(cluster=w290, "CachedData.CD Path"=w288, "CachedData.CD IP"=w284) -> (w289:T4)
                n130 = Build Array (concatenate)(w287, string[] ["Cache.Update", "Object.Initialize", "UI.Override.Hide", "Stream.Disable", "UI.Stream.Disabled", "UI.Log.Enabled", "VS.CheckConnect"]) -> (w286:string[])
              }
              frame True {
                # "User canceled"
              }
            }
          }
          frame "Object.Connected" {
            # "System state is Connected. Get path to required channels and start UDP acquisition if channels found."
            n131 = Unbundle By Name(w319) -> ("CachedData.CD Path"=w301:string, "NIVS.SysDefRoot"=w314:refnum<k24>, "UI.Refs.Cmd"=w312:refnum<vi>)
            n132 = call "UI.Addon.Path.Parse.vi"("Cached Addon Path"=w301) -> ("Addon Path"=w297:string)  [unwired: 6 in, 4 out]
            n133 = call "Workspace.Channels.Create.vi"("CD Path"=w301) -> ("Read Channels"=w317:string[], "Command Channel"=w316:string)  [unwired: 9 in]
            n134 = call "Workspace.CAN.Protocol.Get.vi"("error in (no error)"=w315, "Path"=w297, "NIVS.SysDef Ref"=w314) -> ("error out"=w300:errorcluster, "Diagnostic Protocol"=w313:T10, "NIVS.SysDef Ref out"=w298:refnum<k24>)  [unwired: 6 in]
            n135 = call "Workspace.CAN.TransportProtocol.Get.vi"("error in (no error)"=w300, "Path"=w297, "NIVS.SysDef Ref"=w298) -> ("error out"=w299:errorcluster, "Transport Protocol"=w293:T12)  [unwired: 6 in, 1 out]
            n136 = Not Equal?(x=w293, y=Transport."Diagnostics on IP") -> (x != y?=w294:bool)
            n137 = case shown="\"GMLAN\"" w313 {
              tunnel: [w325 w327 w329] -> w311
              tunnel: [bool[] [TRUE, TRUE, TRUE] bool[] [TRUE, TRUE, TRUE] bool[] [TRUE, TRUE, FALSE]] -> w308
              frame "GMLAN" {
                w325 = T1[] [] items=["None", "Clear Status Channels", "Read All DIDs", "Read All PIDs", "Configure and Start DPIDs", "Stop DPIDs"] ("Disabled Items []")
              }
              frame "KWP-2000", "UDS" {
                w327 = T1[] [enum."Read All PIDs", enum."Configure and Start DPIDs", enum."Stop DPIDs"] items=["None", "Clear Status Channels", "Read All DIDs", "Read All PIDs", "Configure and Start DPIDs", "Stop DPIDs"] ("Disabled Items []")
              }
              frame "User-Defined" {
                w329 = T1[] [enum."Read All DIDs", enum."Read All PIDs", enum."Configure and Start DPIDs", enum."Stop DPIDs"] items=["None", "Clear Status Channels", "Read All DIDs", "Read All PIDs", "Configure and Start DPIDs", "Stop DPIDs"] ("Disabled Items []")
              }
            }
            n138 = Bundle By Name(cluster=w319, "Command.Channel"=w316, "Data.Read"=w317, "Diagnostic Protocol"=w313, "Transport Layer"=w293) -> (w303:T4)
            n139 = property class="Enum (strict)"(reference=w312, error in=w299, "Disabled Items []"=w311) -> (error out=w310:errorcluster)  [unwired: 1 out]
            n140 = property on="Tab Control" class="TabCtl (strict)"(error in=w310) -> (error out=w307:errorcluster, "Pages"=w309:refnum<vi>[])  [unwired: 1 in, 1 out]
            n141 = Build Array (concatenate)(w308, w294) -> (w295:bool[])
            n142 = for {
              tunnel: w309 -> [w323] mode=indexing
              tunnel: w295 -> [w322] mode=indexing
              shift-right: [w320] -> w305
              shift-left: w307 -> [w321]
              n143 = property class="Page"(reference=w323, error in=w321, "PageVis"=w322) -> (error out=w320:errorcluster)  [unwired: 1 out]
            }
            n144 = call "Workspace.UI.DisableState.Set.vi"("Enable?"=TRUE, "error in (no error)"=w305, "State Variables in"=w303) -> ("error out"=w304:errorcluster, "State Variables out"=w302:T4)  [unwired: 7 in]
          }
          frame "Object.Disconnected" {
            n145 = call "Workspace.UI.DisableState.Set.vi"("Enable?"=FALSE, "error in (no error)"=w333, "State Variables in"=w332) -> ("error out"=w330:errorcluster, "State Variables out"=w331:T4)  [unwired: 7 in]
          }
          frame "VS.CheckConnect" {
            n146 = Unbundle By Name(w338) -> ("UI.Refs.Device"=w337:refnum<vi>, "NIVS.Workspace"=w349:T7, "NIVS.SysDefRoot"=w348:refnum<k24>, "CachedData.CD Path"=w347:string)
            n147 = Current VI's Menubar() -> (w350:refnum<k9>)
            n148 = call "UI.Connection.State.Get.vi"("Menu Ref"=w350, "Name Ref"=w337, "error in (no error)"=w346, "Addon Path in"=w347, "NIVS.System Definition Root in"=w348, "NIVS.Workspace Ref in"=w349) -> ("error out"=w345:errorcluster, "Addon Connected?"=w342:bool, "NIVS.System Definition Root out"=w343:refnum<k24>, "NIVS.Workspace Ref out"=w344:T7, "System Definition File"=w336:path)  [unwired: 1 in]
            n149 = case shown="True" w342 {
              tunnel: [w353 w356] -> w341
              tunnel: w340 -> [w352 w355]
              frame True {
                # "Addon connected"
                n150 = Build Array (concatenate)(w352, string[] ["Object.Connected", "Stream.Filter.Read"]) -> (w353:string[])
              }
              frame False {
                # "Addon not connected"
                n151 = Build Array (concatenate)(w355, string[] ["Object.Disconnected", "UI.Stream.Disabled", "Stream.Disable"]) -> (w356:string[])
              }
            }
            n152 = Bundle By Name(cluster=w338, "NIVS.SysDef"=w336, "NIVS.Workspace"=w344, "NIVS.SysDefRoot"=w343, "Addon.Connected?"=w342) -> (w339:T4)
          }
          frame "Object.Exit" {
            # "Stop current loop.  Queue Stop Acq and Exit to UDP loop."
            n153 = Unbundle By Name(w358) -> ("Stream.Qs"=w357:T11)
            n154 = call "Send Host Stream Command Exit.vi"("error in (no error)"=w359, "Q Refs"=w357) -> ("error out"=w360:errorcluster)  [unwired: 9 in]
          }
          frame "Cache.Update" {
            # "Cache any data needing to be permenantly stored with the workspace object."
            n155 = Unbundle By Name(w365) -> ("CachedData.UserEvent"=w363:refnum<user-event>, "CachedData"=w364:T6)
            n156 = Bundle By Name(cluster=T13 {"Operation"=enum."SetCustomData", "Data"=variant} ("event data"), "Data"=w364) -> (w366:T13)
            n157 = Generate User Event(user event=w363, event data cluster=w366) -> ()  [unwired: 2 in, 2 out]
          }
          frame "Channels.Get" {
            # "Get the current slow speed channel values from VeriStand if no pending change, data paths are valid and system state is connected."
            n158 = Unbundle By Name(w375) -> ("UI.Refs"=w370:T5, "Data.PendingChange?"=w371:bool, "Addon.Connected?"=w381:bool, "NIVS.Workspace"=w377:T7, "Data.Read"=w376:string[])  [unwired: 1 out]
            n159 = case shown="False" w381 {
              tunnel: w380 -> [w388 w394]
              tunnel: [w388 w393] -> w372
              tunnel: w377 -> [w387 w392]
              tunnel: [w387 w391] -> w374
              tunnel: w376 -> [w386 w390]
              tunnel: [w383 w389] -> w373
              frame False {
                # "Do Nothing."
                n160 = Array Size(array=w386) -> (size(s)=w385:i32)
                n161 = Initialize Array(0.0 ("element"), w385) -> (w383:dbl[])
              }
              frame True {
                # "Connected & paths valid"
                n162 = call-poly <vilib>:"NI VeriStand - Get Channel Value.vi"("error in (no error)"=w394, "Channels"=w390, "WorkspaceManager in"=w392) -> ("error out"=w393:errorcluster, "Values"=w389:dbl[], "WorkspaceManager out"=w391:T7)  [unwired: 6 in]
              }
            }
            n163 = call "Workspace.UI.Update.vi"("error in (no error)"=w372, "Data.PendingChange?"=w371, "Values"=w373, "UI.Refs"=w370) -> ("error out"=w379:errorcluster)  [unwired: 7 in]
            n164 = Bundle By Name(cluster=w375, "NIVS.Workspace"=w374, "Data.PreviousValues"=w373) -> (w378:T4)
          }
          frame "Channels.Set" {
            # "Set Channels if data paths are valid and system state is connected and there is a change in the data value."
            n165 = Unbundle By Name(w402) -> ("Addon.Connected?"=w398:bool, "NIVS.Workspace"=w397:T7, "Command.Channel"=w395:string, "UI.Refs"=w396:T5)
            n166 = case shown="False" w398 {
              tunnel: w404 -> [w407 w409]
              tunnel: [w407 w415] -> w403
              tunnel: w397 -> [w406 w414]
              tunnel: [w406 w413] -> w399
              tunnel: w395 -> [_ w412]
              tunnel: w396 -> [_ w410]
              frame False {
                # "Do nothing"
              }
              frame True {
                # "Connected & paths valid"
                n167 = call "Workspace.UI.Pull.vi"("error in (no error)"=w409, "UI.Refs"=w410) -> ("error out"=w408:errorcluster, "Value"=w411:dbl)  [unwired: 8 in]
                n168 = call-poly <vilib>:"NI VeriStand - Set Channel Value.vi"("error in (no error)"=w408, "Value"=w411, "Channel"=w412, "WorkspaceManager in"=w414) -> ("error out"=w415:errorcluster, "WorkspaceManager out"=w413:T7)  [unwired: 6 in]
              }
            }
            n169 = Bundle By Name(cluster=w402, "Data.PendingChange?"=FALSE ("Pending Change?"), "NIVS.Workspace"=w399) -> (w401:T4)
          }
          frame "UI.Override.Hide" {
            # "Reset slow speed channel displayed values."
            n170 = Unbundle By Name(w422) -> ("UI.Refs.DTC"=w421:refnum<vi>, "UI.Refs.Status"=w420:refnum<vi>, "UI.Refs.Failure"=w419:refnum<vi>)
            n171 = Build Array(w421, w420, w419) -> (w418:refnum<vi>[])
            n172 = for {
              tunnel: w418 -> [w428] mode=indexing
              shift-right: [w426] -> w416
              shift-left: w417 -> [w427]
              n173 = property class="DigNum (strict)"(reference=w428, error in=w427, "Visible"=FALSE, "Value"=u32 0) -> (error out=w426:errorcluster)  [unwired: 1 out]
            }
          }
          frame "UI.Override.Show" {
            # "Reset slow speed channel displayed values."
            n174 = Unbundle By Name(w435) -> ("UI.Refs.DTC"=w434:refnum<vi>, "UI.Refs.Status"=w433:refnum<vi>, "UI.Refs.Failure"=w432:refnum<vi>)
            n175 = Build Array(w434, w433, w432) -> (w431:refnum<vi>[])
            n176 = for {
              tunnel: w431 -> [w440] mode=indexing
              shift-right: [w438] -> w429
              shift-left: w430 -> [w439]
              n177 = property class="DigNum (strict)"(reference=w440, error in=w439, "Visible"=TRUE) -> (error out=w438:errorcluster)  [unwired: 1 out]
            }
          }
          frame "UI.Stream.Enabled" {
            n178 = call "UI.Stream.Enable.vi"("error in (no error)"=w442, "State Variables in"=w441) -> ("error out"=w443:errorcluster)  [unwired: 9 in]
          }
          frame "UI.Log.Enabled" {
            w445 = T20."Disabled and Grayed Out" ("Disabled")
            n179 = Unbundle By Name(w457) -> ("UI.Refs.Type Filter"=w450:refnum<vi>, "UI.Refs.Filter IDs"=w449:refnum<vi>, "UI.Refs.Direction Filter"=w448:refnum<vi>, "UI.Refs.Reset Filter"=w453:refnum<vi>, "UI.Refs.Filter Location"=w456:refnum<vi>)
            n180 = property class="Bool (strict)"(reference=w456, error in=w455, "DisabledEnum"=w445) -> (error out=w454:errorcluster, "Value"=w452:bool)  [unwired: 1 out]
            n181 = Build Array(w450, w449, w448) -> (w447:refnum<vi>[])
            n182 = property class="Bool"(reference=w453, error in=w454, "DisabledEnum"=w445) -> (error out=w451:errorcluster)  [unwired: 1 out]
            n183 = case shown="False" w452 {
              tunnel: w451 -> [w461 w467]
              tunnel: w447 -> [w462 _]
              tunnel: [w460 w467] -> w446
              tunnel: w445 -> [w459 _]
              frame False {
                n184 = for {
                  tunnel: w462 -> [w466] mode=indexing
                  shift-right: [w464] -> w460
                  shift-left: w461 -> [w465]
                  tunnel: w459 -> [w463]
                  n185 = property class="Ctl"(reference=w466, error in=w465, "DisabledEnum"=w463) -> (error out=w464:errorcluster)  [unwired: 1 out]
                }
              }
              frame True {
              }
            }
          }
          frame "UI.Stream.Disabled" {
            n186 = call "UI.Stream.Disable.vi"("error in (no error)"=w469, "State Variables in"=w470) -> ("error out"=w468:errorcluster)  [unwired: 9 in]
          }
          frame "UI.Log.Disabled" {
            w472 = T20."Enabled" ("Disabled")
            n187 = Unbundle By Name(w483) -> ("UI.Refs.Type Filter"=w477:refnum<vi>, "UI.Refs.Filter IDs"=w476:refnum<vi>, "UI.Refs.Direction Filter"=w475:refnum<vi>, "UI.Refs.Reset Filter"=w479:refnum<vi>, "UI.Refs.Filter Location"=w482:refnum<vi>)
            n188 = property class="Bool (strict)"(reference=w482, error in=w481, "DisabledEnum"=w472) -> (error out=w480:errorcluster)  [unwired: 1 out]
            n189 = Build Array(w477, w476, w475) -> (w474:refnum<vi>[])
            n190 = property class="Bool"(reference=w479, error in=w480, "DisabledEnum"=w472) -> (error out=w478:errorcluster)  [unwired: 1 out]
            n191 = for {
              tunnel: w474 -> [w488] mode=indexing
              shift-right: [w486] -> w473
              shift-left: w478 -> [w487]
              tunnel: w472 -> [w485]
              n192 = property class="Ctl"(reference=w488, error in=w487, "DisabledEnum"=w485) -> (error out=w486:errorcluster)  [unwired: 1 out]
            }
          }
          frame "Raw.Send" {
            # "Reset slow speed channel displayed values."
            n193 = Unbundle By Name(w503) -> ("CachedData.CD IP"=w492:string, "CachedData.CD Path"=w490:string)
            n194 = call "UI.Addon.Path.Parse.vi"("Cached Addon Path"=w490) -> ("Addon Name"=w489:string)  [unwired: 6 in, 4 out]
            n195 = Bundle By Name(cluster=cluster{"cmd":u8[], "require response?":bool} {"cmd"=[], "require response?"=TRUE} ("Cmd"), "cmd"="Raw Cmd", "require response?"="Response Required?") -> (w501:cluster{"cmd":u8[], "require response?":bool})
            n196 = call "Connect.vi"("Addon Name"=w489, "Address"=w492) -> ("error out"=w498:errorcluster, "Ref out"=w504:T21)  [unwired: 8 in]
            n197 = call "PassThru.vi"("error in (no error)"=w498, "timeout ms (1000)"=2500, "Cmd"=w501, "Ref"=w504) -> ("error out"=w497:errorcluster, "Resp"=w496:T25, "Ref out"=w505:T21)  [unwired: 5 in]
            n198 = Unbundle By Name(w496) -> ("resp"=→"Raw Resp":u8[], "error code"=→"Raw Error Byte":u8, "error out"=→"Raw VeriStand Error":errorcluster)
            n199 = call "Disconnect.vi"("error in"=w497, "Ref"=w505) -> ()  [unwired: 9 in, 1 out]
          }
          frame "Raw.Clear" {
            n200 = local write "Raw Cmd"(u8[] [] ("Cmd")) -> ()
          }
          frame "DTC.Read" {
            # "Reset slow speed channel displayed values."
            n201 = Unbundle By Name(w535) -> ("CachedData.CD IP"=w533:string, "CachedData.CD Path"=w534:string)
            n202 = Bundle By Name(cluster=T14 {"Extension"=0, "Mask"=0, "Mode/Status"=0, "Byte Lengths"={"Override"=FALSE, "DTC"=0, "Status"=0, "Failure"=0}} ("Options (KWP/UDS Only)"), "Extension"="Extension", "Mask"="Mask", "Mode/Status"="Mode", "Byte Lengths.Override"="Override Byte Lengths", "Byte Lengths.DTC"="DTC", "Byte Lengths.Status"="Status", "Byte Lengths.Failure"="Failure") -> (w527:T14)
            n203 = call "UI.Addon.Path.Parse.vi"("Cached Addon Path"=w534) -> ("Addon Name"=w512:string)  [unwired: 6 in, 4 out]
            n204 = call "Connect.vi"("Addon Name"=w512, "Address"=w533) -> ("error out"=w531:errorcluster, "Ref out"=w532:T21)  [unwired: 8 in]
            n205 = call "ReadDTCs.vi"("error in (no error)"=w531, "timeout ms (1000)"=2500, "Options (KWP/UDS Only)"=w527, "Ref"=w532) -> ("error out"=w530:errorcluster, "Active DTCs"=w517:T26[], "Ref out"=w529:T21)  [unwired: 5 in]
            n206 = call "Disconnect.vi"("error in"=w530, "Ref"=w529) -> ("error out"=w522:errorcluster)  [unwired: 9 in]
            n207 = control-ref of="DTCs"() -> (w514:refnum<vi>)
            n208 = call <vilib>:"Simple Error Handler.vi"("error in (no error)"=w522) -> ()  [unwired: 4 in, 5 out]
            n209 = call "Workspace.DTC.Update.vi"("Hex"="Hex", "error in"=w515, "Active DTCs"=w517, "DTCs"=w514) -> ("error out"=w513:errorcluster)  [unwired: 7 in]
          }
          frame "Stream.Enable" {
            n210 = Unbundle By Name(w542) -> ("Stream.Qs"=w539:T11, "CachedData.CD IP"=w540:string, "CachedData.CD Path"=w546:string, "NIVS.SysDef"=w538:path)
            n211 = Strip Path(path=w538) -> (stripped path=w537:path)  [unwired: 1 out]
            n212 = call "UI.Addon.Path.Parse.vi"("Cached Addon Path"=w546) -> ("Addon Name"=w541:string)  [unwired: 6 in, 4 out]
            n213 = call "Send Host Stream Command Start.vi"("Project Folder"=w537, "error in (no error)"=w544, "Addon"=w541, "Target IP Address"=w540, "Q Refs"=w539) -> ("error out"=w543:errorcluster)  [unwired: 6 in]
          }
          frame "Stream.Filter.Send" {
            n214 = Unbundle By Name(w559) -> ("CachedData.CD IP"=w557:string, "CachedData.CD Path"=w560:string)
            n215 = local read "Direction Filter"() -> (w548:T3)
            n216 = local read "Type Filter"() -> (w549:T2)
            n217 = local read "Filter IDs"() -> (w550:string)
            n218 = call "Convert Filter IDs String to Array.vi"("Filter IDs"=w550) -> ("Filter IDs"=w547:u32[])  [unwired: 10 in]
            n219 = call "UI.Addon.Path.Parse.vi"("Cached Addon Path"=w560) -> ("Addon Name"=w558:string)  [unwired: 6 in, 4 out]
            n220 = Bundle By Name(cluster=T16 {"ID Filters"=[], "Direction Filter"=enum."Tx/Rx", "Type Filter"=enum."All"} ("IDs"), "Direction Filter"=w548, "Type Filter"=w549, "ID Filters"=w547) -> (w551:T16)
            n221 = call "Connect.vi"("Addon Name"=w558, "Address"=w557) -> ("error out"=w554:errorcluster, "Ref out"=w553:T21)  [unwired: 8 in]
            n222 = call "SetStreamingFilter.vi"("error in (no error)"=w554, "IDs"=w551, "Ref"=w553) -> ("error out"=w562:errorcluster, "Ref out"=w561:T21)  [unwired: 7 in]
            n223 = call "Disconnect.vi"("error in"=w562, "Ref"=w561) -> ("error out"=w555:errorcluster)  [unwired: 9 in]
            n224 = call <vilib>:"Simple Error Handler.vi"("error in (no error)"=w555) -> ()  [unwired: 4 in, 5 out]
          }
          frame "Stream.Filter.Clear" {
            n225 = Unbundle By Name(w571) -> ("CachedData.CD IP"=w569:string, "CachedData.CD Path"=w572:string)
            n226 = call "UI.Addon.Path.Parse.vi"("Cached Addon Path"=w572) -> ("Addon Name"=w570:string)  [unwired: 6 in, 4 out]
            n227 = call "Connect.vi"("Addon Name"=w570, "Address"=w569) -> ("error out"=w566:errorcluster, "Ref out"=w565:T21)  [unwired: 8 in]
            n228 = call "SetStreamingFilter.vi"("error in (no error)"=w566, "IDs"=T16 {"ID Filters"=[], "Direction Filter"=enum."Tx/Rx", "Type Filter"=enum."All"}, "Ref"=w565) -> ("error out"=w574:errorcluster, "Ref out"=w573:T21)  [unwired: 7 in]
            n229 = call "Disconnect.vi"("error in"=w574, "Ref"=w573) -> ("error out"=w567:errorcluster)  [unwired: 9 in]
            n230 = call <vilib>:"Simple Error Handler.vi"("error in (no error)"=w567) -> ()  [unwired: 4 in, 5 out]
          }
          frame "Stream.Filter.Reset" {
            n231 = Unbundle By Name(w588) -> ("CachedData.CD IP"=w586:string, "CachedData.CD Path"=w589:string)
            n232 = call "UI.Addon.Path.Parse.vi"("Cached Addon Path"=w589) -> ("Addon Name"=w587:string)  [unwired: 6 in, 4 out]
            n233 = call "Connect.vi"("Addon Name"=w587, "Address"=w586) -> ("error out"=w583:errorcluster, "Ref out"=w582:T21)  [unwired: 8 in]
            n234 = call "ResetStreamingFilter.vi"("error in (no error)"=w583, "Ref"=w582) -> ("error out"=w591:errorcluster, "IDs"=w578:T16, "Ref out"=w590:T21)  [unwired: 7 in]
            n235 = local write "Host Filter"(FALSE ("Host Filter")) -> ()
            n236 = Unbundle By Name(w578) -> ("ID Filters"=w577:u32[], "Direction Filter"=w580:T3, "Type Filter"=w579:T2)
            n237 = call "Disconnect.vi"("error in"=w591, "Ref"=w590) -> ("error out"=w584:errorcluster)  [unwired: 9 in]
            n238 = call <vilib>:"Simple Error Handler.vi"("error in (no error)"=w584) -> ()  [unwired: 4 in, 5 out]
            n239 = call "Convert Filter IDs Array to String.vi"("Filter IDs"=w577) -> ("Filter IDs"=w576:string)  [unwired: 10 in]
            n240 = local write "Filter IDs"(w576) -> ()
            n241 = local write "Direction Filter"(w580) -> ()
            n242 = local write "Type Filter"(w579) -> ()
          }
          frame "Stream.Filter.Read" {
            n243 = Unbundle By Name(w602) -> ("CachedData.CD IP"=w600:string, "CachedData.CD Path"=w603:string)
            n244 = call "UI.Addon.Path.Parse.vi"("Cached Addon Path"=w603) -> ("Addon Name"=w601:string)  [unwired: 6 in, 4 out]
            n245 = call "Connect.vi"("Addon Name"=w601, "Address"=w600) -> ("error out"=w606:errorcluster, "Ref out"=w607:T21)  [unwired: 8 in]
            n246 = call "GetStreamingFilter.vi"("error in (no error)"=w606, "Ref"=w607) -> ("error out"=w605:errorcluster, "IDs"=w597:T16, "Ref out"=w604:T21)  [unwired: 7 in]
            n247 = Unbundle By Name(w597) -> ("ID Filters"=w594:u32[], "Direction Filter"=w596:T3, "Type Filter"=w595:T2)
            n248 = call "Disconnect.vi"("error in"=w605, "Ref"=w604) -> ("error out"=w598:errorcluster)  [unwired: 9 in]
            n249 = call <vilib>:"Simple Error Handler.vi"("error in (no error)"=w598) -> ()  [unwired: 4 in, 5 out]
            n250 = call "Convert Filter IDs Array to String.vi"("Filter IDs"=w594) -> ("Filter IDs"=w593:string)  [unwired: 10 in]
            n251 = local write "Filter IDs"(w593) -> ()
            n252 = local write "Direction Filter"(w596) -> ()
            n253 = local write "Type Filter"(w595) -> ()
          }
          frame "Stream.Table.GoUp" {
            n254 = Unbundle By Name(w613) -> ("UI.Refs.Table Control"=w611:refnum<vi>)
            n255 = property class="Tbl (strict)"(reference=w611, error in=w609, "Index Values"=T17 {"Row"=0, "Column"=0}) -> (error out=w610:errorcluster)  [unwired: 1 out]
          }
          frame "Stream.Disable" {
            n256 = Unbundle By Name(w618) -> ("Stream.Qs"=w617:T11)
            n257 = call "Send Host Stream Command Stop.vi"("error in (no error)"=w615, "Q Refs"=w617) -> ("error out"=w616:errorcluster)  [unwired: 9 in]
          }
        }
      }
      frame Error {
        # "Handle Errors."
        n258 = Unbundle By Name(w622) -> ("code"=w626:i32)
        n259 = Equal?(x=-307654, y=w626) -> (x = y?=w624:bool)
        n260 = Select(t=errorcluster {"status"=FALSE, "code"=0, "source"=""}, s=w624, f=w622) -> (s? t:f=w621:errorcluster)
        n261 = call <vilib>:"Simple Error Handler.vi"("error in (no error)"=w621) -> ("error out"=w627:errorcluster)  [unwired: 4 in, 4 out]
        n262 = call <vilib>:"Clear Errors.vi"("error in (no error)"=w627) -> ("error out"=w620:errorcluster)  [unwired: 5 in, 1 out]
      }
    }
  }
  n263 = while {
    tunnel: w10 -> [w656]
    tunnel: w9 -> [w655]
    tunnel: [w648] -> w8
    stop <- w647 stop-if-true
    n264 = Unbundle By Name(w655) -> ("UI.Refs.CAN State"=w652:refnum<vi>, "Stream.Qs"=w654:T11)
    n265 = call "Convert Filter IDs String to Array.vi"("Filter IDs"="Filter IDs") -> ("Filter IDs"=w630:u32[])  [unwired: 10 in]
    n266 = Bundle By Name(cluster=T27 {"Host Filter"=FALSE, "Filter Parameters"={"ID Filters"=[], "Direction Filter"=enum."Tx/Rx", "Type Filter"=enum."All"}, "Sort By ID"=FALSE, "Pause"=FALSE, "Clear History"=FALSE, "Log"=FALSE} ("Host Parameters"), "Clear History"="Clear History", "Pause"="Pause", "Sort By ID"="Sort By ID", "Filter Parameters.Direction Filter"="Direction Filter", "Filter Parameters.Type Filter"="Type Filter", "Host Filter"="Host Filter", "Log"="Log", "Filter Parameters.ID Filters"=w630) -> (w642:T27)
    n267 = call "Main Engine Host Stream.vi"("error in (no error)"=w656, "Host Parameters"=w642, "Q Refs"=w654) -> ("error out"=w653:errorcluster, "Exit"=w647:bool, "Stream"=w651:T28)  [unwired: 6 in]
    n268 = Unbundle By Name(w651) -> ("Bus Warning"=w650:bool, "Connected"=→"Stream Connected":bool, "Bus Status"=w641:string, "Log Status"=w637:string, "Bus Data Update"=w636:bool, "Bus Data"=w635:string[][])
    n269 = property class="Str"(reference=w652, error in=w653, "Blinking"=w650) -> (error out=w648:errorcluster)  [unwired: 1 out]
    n270 = Concatenate Strings(w641, "\r\n", w637) -> (→"Status":string)
    n271 = case shown="True" w636 {
      tunnel: w635 -> [_ w657]
      frame False {
      }
      frame True {
        "Table Control" <- w657
      }
    }
  }
  n272 = flat-sequence {
    tunnel: w36 -> [w658]
    tunnel: w8 -> [_]
    frame #0 {
      n273 = call "Workspace.Close.vi"("State Variables in"=w658) -> ()  [unwired: 11 in]
    }
    frame #1 {
      n274 = invoke class="VI" method="FP.Close"() -> ()  [unwired: 3 in, 3 out]
    }
  }
